vi "VIH Project Tree - Get PolyVI Instance VIs.vi"(5 "Project Tree":T1, 7 "Items Array":T3[](array[typedef]), 8 "error in":errorcluster, 10 "Item Items Data":T2(array[cluster]), 11 "Item Parent Tags":string[](array[string])) -> (0 "error out":errorcluster, 2 "Item Items Data out":T2(array[cluster]), 3 "Item Parent Tags out":string[](array[string]))   [LabVIEW 2014]
doc: "::: VI Helpeks :::\nCopyright (c) 2000-2026 Konstantin Shifershteyn. All rights reserved."
uses:
  _VIH HelpGen - Palette.llb/VIH HelpGen Typedef - Palette - Item Info Cluster.ctl
  _VIH HelpGen - Palette.llb/VIH HelpGen Typedef - Palette - Item Type Enum.ctl
  VIH Project Tree Typedef - Tree Refnum.ctl
  VIH Project Tree Typedef - Tree Item Type.ctl
panel:
  # "VI Helpeks\nCopyright (c) 2012-2026 Konstantin Shifershteyn"
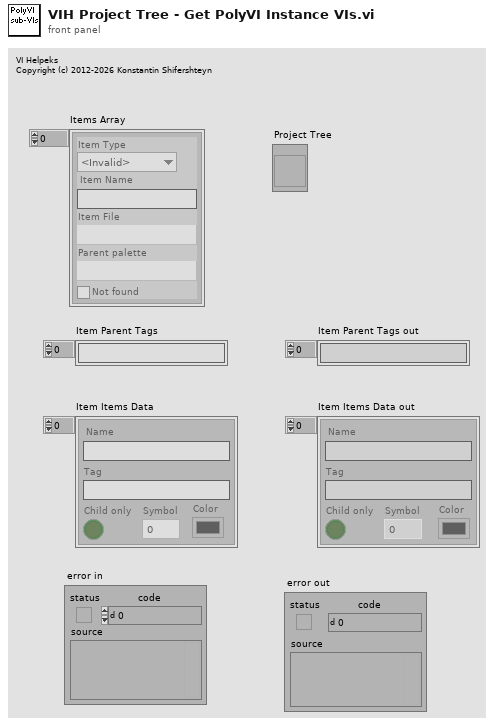
[diagram p1: front panel]
types:
  T1 = typedef "VIH Project Tree Typedef - Tree Refnum.ctl" = refnum<vi>
  T2 = cluster{"Name":string, "Tag":string, "Child only":bool, "Symbol":i32, "Color":u32}[]
  T3 = typedef "VIH HelpGen Typedef - Palette - Item Info Cluster.ctl" = cluster{"Item Type":T4, "Item Name":string, "Item File":path, "Parent palette":path, "Not found":bool}
  T4 = typedef "VIH HelpGen Typedef - Palette - Item Type Enum.ctl" = enum32{"<Invalid>", "<unknown>", "VI", "Menu", "LV Func", "Express VI", "Poly VI", "CTL", "HTML"}
  T5 = typedef "VIH Project Tree Typedef - Tree Item Type.ctl" = enum32{"<Invalid>", "Project", "Proj Files", "Proj Rules", "File Group", "Rule Group", "Any File", "LV Func", ".mnu", ".mnu (dyn)", ".vi", ".vi (dyn)", ".vit", ".vit (dyn)", ".ctl", ".ctl (dyn)", ".ctt", ".ctt (dyn)", "polyVI", "polyVI (dyn)", "expVI", "expVI (dyn)", "HTML", "PolyVI Inst"}
  T6 = cluster{"Name":string, "Tag":string, "Child only":bool, "Symbol":i32, "Color":u32}
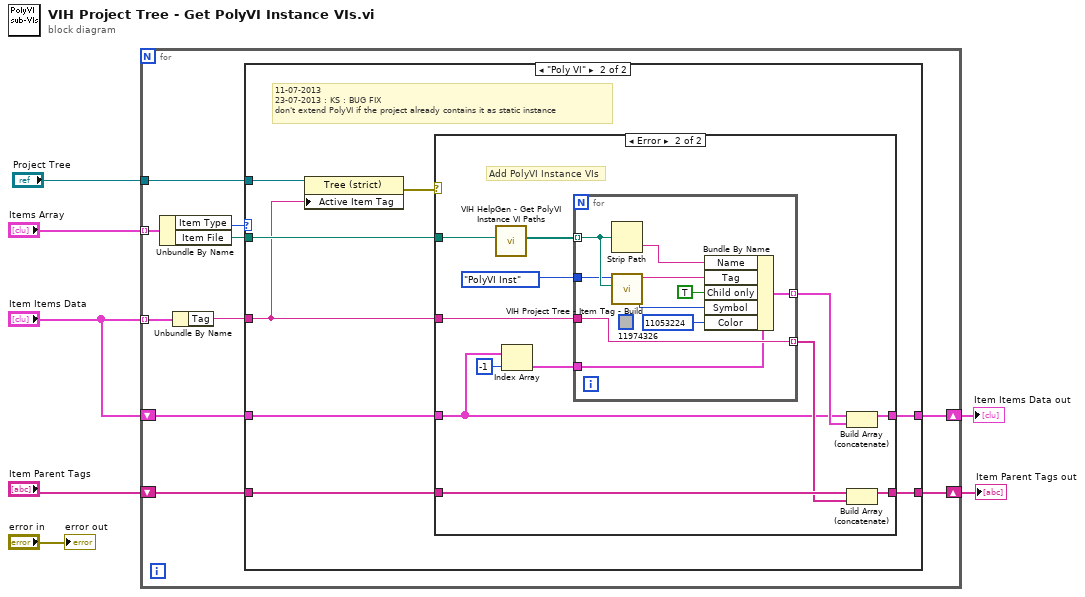
[diagram p0: block diagram]
diagram:
  n1 = for {
    tunnel: "Items Array" -> [w17] mode=indexing
    tunnel: "Item Items Data" -> [w9] mode=indexing
    shift-right: [w11] -> w4
    shift-left: "Item Items Data" -> [w14]
    shift-right: [w12] -> w3
    shift-left: "Item Parent Tags" -> [w13]
    tunnel: "Project Tree" -> [w10]
    n2 = Unbundle By Name(w17) -> ("Item Type"=w16:T4, "Item File"=w15:path)
    n3 = Unbundle By Name(w9) -> ("Tag"=w8:string)
    n4 = case shown="\"Poly VI\"" w16 {
      tunnel: w15 -> [_ w23]
      tunnel: w14 -> [w19 w24]
      tunnel: w13 -> [w18 w27]
      tunnel: [w18 w26] -> w12
      tunnel: [w19 w25] -> w11
      tunnel: w10 -> [_ w22]
      tunnel: w8 -> [_ w21]
      frame Default {
      }
      frame "Poly VI" {
        # "11-07-2013\n23-07-2013 : KS : BUG FIX\ndon't extend PolyVI if the project already contains it as static instance"
        n5 = property class="Tree (strict)"(reference=w22, "Active Item Tag"=w21) -> (error out=w20:errorcluster)  [unwired: 1 in, 1 out]
        n6 = case shown="Error" w20 {
          tunnel: w21 -> [_ w30]
          tunnel: w27 -> [w29 w38]
          tunnel: [w29 w36] -> w26
          tunnel: [w28 w35] -> w25
          tunnel: w24 -> [w28 w33]
          tunnel: w23 -> [_ w31]
          frame No Error {
            # "There is a static file with this tag in the tree.\n\n*) static files have constant tree tags"
          }
          frame Error {
            # "Add PolyVI Instance VIs"
            n7 = call "VIH HelpGen - Get PolyVI Instance VI Paths.vi"("VI Path"=w31) -> ("Instance VI Paths"=w41:path[])  [unwired: 8 in, 2 out]
            n8 = Index Array(array=w33, index=-1) -> (element=w32:T6)
            n9 = for {
              tunnel: w41 -> [w49] mode=indexing
              tunnel: VIH_Project_Tree_Typedef_-_Tree_Item_Type."PolyVI Inst" ("Item Type") -> [w48]
              tunnel: [w45] -> w39 mode=indexing
              tunnel: [w44] -> w37 mode=indexing
              tunnel: w30 -> [w44]
              tunnel: w32 -> [w43]
              (unwired) u32 11974326
              n10 = Strip Path(path=w49) -> (name=w47:string)  [unwired: 1 out]
              n11 = call "VIH Project Tree - Item Tag - Build.vi"("Item File Path"=w49, "Item Type"=w48) -> ("Tree Item Symbol"=w51:i32, "Tree Item Tag"=w50:string)  [unwired: 8 in]
              n12 = Bundle By Name(cluster=w43, "Name"=w47, "Tag"=w50, "Child only"=TRUE, "Symbol"=w51, "Color"=u32 11053224) -> (w45:T6)
            }
            n13 = Build Array (concatenate)(w33, w39) -> (w35:T2)
            n14 = Build Array (concatenate)(w38, w37) -> (w36:string[])
          }
        }
      }
    }
  }
  "Item Items Data out" <- w4
  "Item Parent Tags out" <- w3
  "error out" <- "error in"
